vi "PicoScope2000aSetRapidSegments.vi"(5 "RapidBlock":bool, 7 "nSegments":T1 format="%.4p", 8 "error in (no error)":errorcluster, 11 "handle in":i16) -> (0 "error out":errorcluster, 3 "handle out":i16, 6 "nCaptures":u64)   [LabVIEW 2009]
doc: "Calls ps2000aMemorySegments, and ps2000aSetNoOfCaptures"
uses:
  ps2000a.dll
  shared/nSegments.ctl
panel:
  out "nMaxSamples":u64
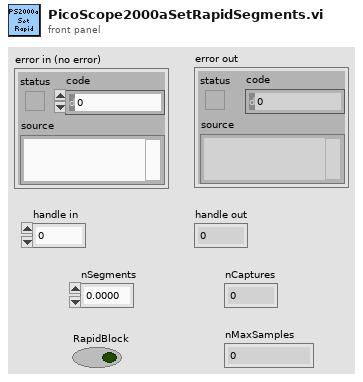
[diagram p1: front panel]
types:
  T1 = typedef "nSegments.ctl" = u64
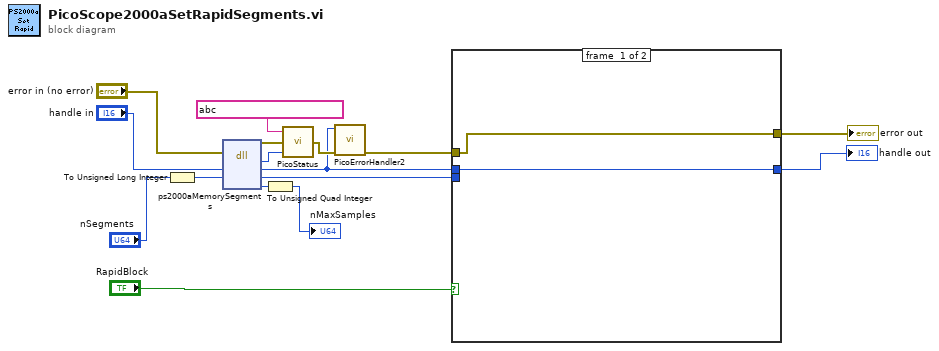
[diagram p0: block diagram]
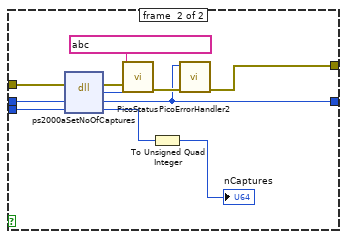
[diagram p2: hidden frame]
diagram:
  n1 = To Unsigned Long Integer(number="nSegments") -> (unsigned 32bit integer=w4:u32)
  n2 = dll-call lib="ps2000a.dll" fn="ps2000aMemorySegments" ("ps3000.dll:_ps3000_open_unit@0")(error in="error in (no error)", "handle"="handle in", "nSegments"=w4) -> (error out=w15:errorcluster, "PICO_STATUS"=w16:u32, "handle"=w11:i16, "nSegments"=w13:u32, "nMaxSamples"=w2:i32)  [unwired: 3 in, 1 out]
  n3 = To Unsigned Quad Integer(1:w2) -> (0:→"nMaxSamples":u64)
  n4 = call "PicoStatus.vi"("PICO STATUS"=w16, "error in"=w15, "source"=string ?) -> ("error out"=w12:errorcluster)
  n5 = call "PicoErrorHandler2.vi"("error in (no error)"=w12, "handle In"=w11) -> ("error out"=w10:errorcluster)  [unwired: 9 in]
  n6 = case shown="True" "RapidBlock" {
    tunnel: w13 -> [_ w29]
    tunnel: w11 -> [w17 w26]
    tunnel: w10 -> [w18 w23]
    tunnel: [w18 w22] -> w7
    tunnel: [w17 w21] -> w6
    frame #0 {
    }
    frame #1 {
      n7 = dll-call lib="ps2000a.dll" fn="ps2000aSetNoOfCaptures" ("ps3000.dll:_ps3000_open_unit@0")(error in=w23, "handle"=w26, "nCaptures"=w29) -> (error out=w28:errorcluster, "PICO_STATUS"=w24:u32, "handle"=w21:i16, "nCaptures"=w20:u32)  [unwired: 2 in, 1 out]
      n8 = call "PicoStatus.vi"("PICO STATUS"=w24, "error in"=w28, "source"=string ?) -> ("error out"=w25:errorcluster)
      n9 = To Unsigned Quad Integer(1:w20) -> (0:→"nCaptures":u64)
      n10 = call "PicoErrorHandler2.vi"("error in (no error)"=w25, "handle In"=w21) -> ("error out"=w22:errorcluster)  [unwired: 9 in]
    }
  }
  "error out" <- w7
  "handle out" <- w6
